vi "Replace Dependency.vi"(6 "New SubVI":path, 8 "error in":errorcluster, 9 "SubVI":string, 10 "VI Path":path, 11 "ILV File Creator in":refnum<class "ILV File Creator.lvclass">) -> (0 "error out":errorcluster, 3 "ILV File Creator out":refnum<class "ILV File Creator.lvclass">)   [LabVIEW 2026, in "ILV File Creator.lvclass"]
doc: "This VI will open a reference to the provided VI path, traverse objects and replace the specified SubVI by the new SubVI."
uses:
  ILV File Creator.lvclass
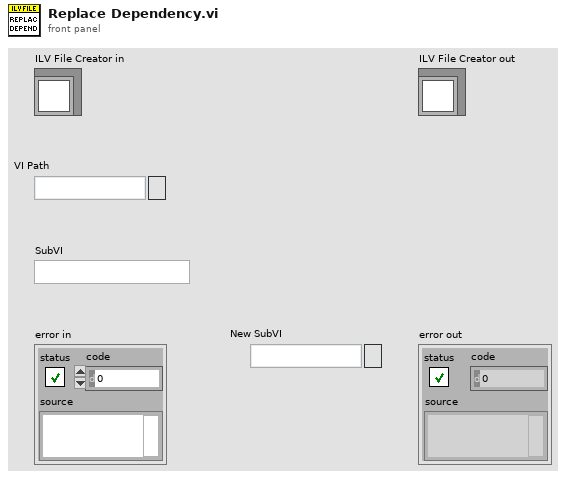
[diagram p1: front panel]
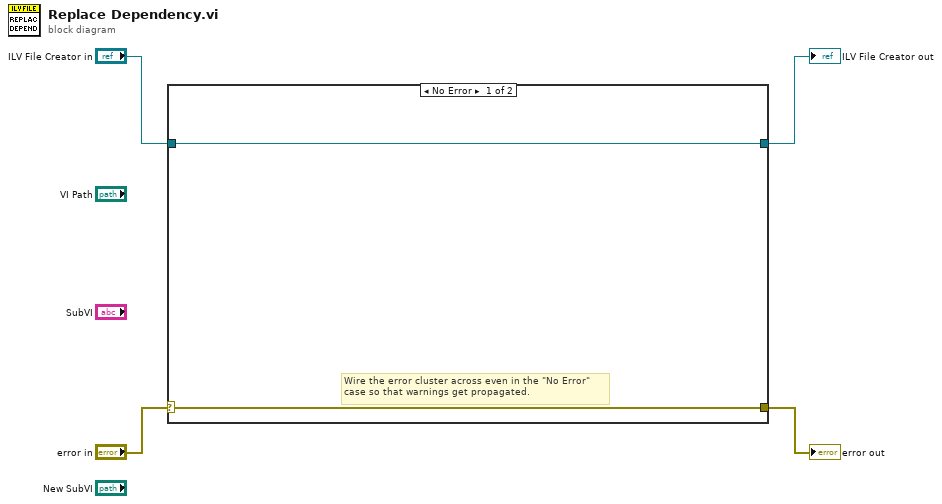
[diagram p0: block diagram]
diagram:
  n1 = case shown="No Error" "error in" {
    selector: "error in" -> [w6 w8]
    tunnel: [w6 w8] -> w3
    tunnel: [w5 w7] -> w1
    tunnel: "ILV File Creator in" -> [w5 w7]
    frame No Error {
      # "Wire the error cluster across even in the \"No Error\"\ncase so that warnings get propagated."
    }
    frame Error {
    }
  }
  "error out" <- w3
  "ILV File Creator out" <- w1
